vi "Software.Service.SNDB Communication Wrapper.vi"(0 "Log In Data":cluster{"Username":string, "Password":string}, 1 "Command":T1, 2 "Verify value":bool, 3 "File Path":string, 5 "Serial Number":string, 9 "Id(handle)":string, 11 "Error In (no error)":errorcluster, 12 "state":string, 13 "value":string) -> (4 "Operation Successful?":bool, 6 "UUT_Type":string, 10 "MAC_addresses":cluster{"MAC":string, "Status":string}[](array[cluster]), 15 "Error Out":errorcluster)   [LabVIEW 2026, in "Connect_to_SNDB_library.lvlib"]
uses:
  Connect_to_SNDB_library.lvlib
  Software.Service.SNDB Communication Wrapper Command.ctl
  Libray.Connect_to_SNDB_Command.ctl
  BB115/LabVIEW/Additional Libraries/Connect to SNDB Library.lvlibp/LabVIEW.Library/Libray.Connect_to_SNDB_Command.ctl
  <vilib>/JDP Science/JSONtext/Next JSON Value.vi
  <vilib>/JDP Science/JSONtext/String Subset.vi
  <vilib>/JDP Science/JSONtext/support/Strip Quotes and Unescape.vi
  <vilib>/JDP Science/JSONtext/Parsing/Advance past next JSON Value (inlined COPY).vi
  <vilib>/JDP Science/JSONtext/support/Unescape JSON string.vi
  <vilib>/JDP Science/JSONtext/Parsing/Advance past whitespace.vi
  <vilib>/JDP Science/JSONtext/Parsing/Advance past String.vi
  <vilib>/JDP Science/JSONtext/Parsing/Advance past Number.vi
  <vilib>/JDP Science/JSONtext/Parsing/Advance past Line Ending.vi
  <vilib>/JDP Science/JSONtext/Parsing/Parse Full Path or Item Name.vi
  <vilib>/JDP Science/JSONtext/Parsing/Advance past Array.vi
  <vilib>/JDP Science/JSONtext/Parsing/Advance past Object.vi
  <vilib>/JDP Science/JSONtext/support/Error Cluster From Code.vi
  <vilib>/JDP Science/JSONtext/Offset/Find Item Locations by Path.vi
  <vilib>/JDP Science/JSONtext/JSONtext.lvlib
  BB115/LabVIEW/Additional Libraries/Connect to SNDB Library.lvlibp
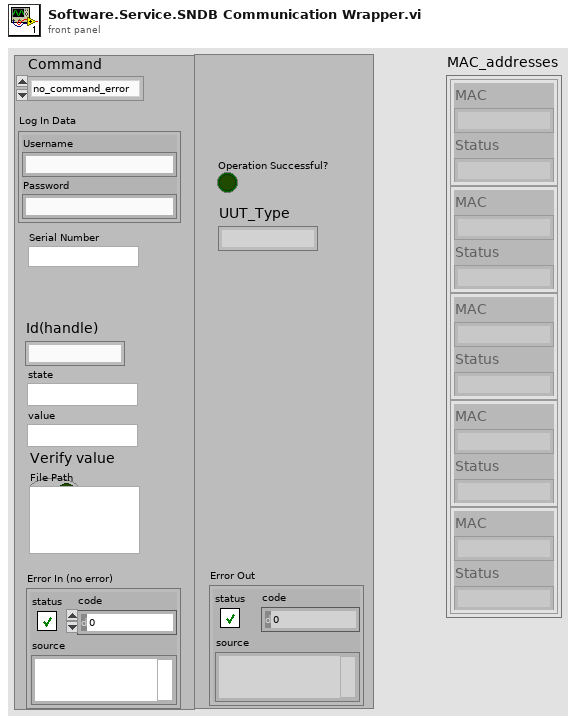
[diagram p1: front panel]
types:
  T1 = typedef "Connect_to_SNDB_library.lvlib/Software.Service.SNDB Communication Wrapper Command.ctl" = enum16{"no_command_error", "Initialize_Components_Login_Create_Token", "Get_UUT_Type", "Update steps", "Upload_PDF_Report", "Revoke_Token_Deinitialize_Components", "Reserve_MAC_addresses_for_a_Serial_Number", "Mark_a_reserved_MAC_address_as_flashed", "Get_all_MAC_addresses_for_a_Serial_Number", "Get_data_of_a_step"}
  T2 = typedef "Connect_to_SNDB_library.lvlib/Libray.Connect_to_SNDB_Command.ctl" = enum16{"No command", "Initialize HTTPS", "Authentication: Creat a token", "Authentication: Get all tokens", "Authentication: Revoke the token", "Label: Creat a label configuration", "Label: Get all configured labels", "Label: Update the label configuration", "Label: Delete the label configuration", "Label: Creat a colour ribbon", "Label: Update the colour ribbon", "Label: Get all colour ribbons", "Label: Delete the colour ribbon", "Label: Creat a label tape", "Label: Update the label tape", "Label: Get all label tapes", "Label: Delete the label tape", "Label: Get all label parameters", "Product: Get all product informations", "Product: Get all reading steps", "Seriennummer: Update the info text", "Seriennummer: Set all step states open", "Seriennummer: Update step states", "Seriennummer: Get data and steps", "Seriennummer: Get all label configurations", "Seriennummer: Create a text report(Prüfbericht)", "Seriennummer: Get the text report(Prüfbericht)", "Seriennummer: Delete the text report(Prüfbericht)", "Seriennummer: Upload a document(txt file)", "Seriennummer: Get the document", "Seriennummer: Get the document thumbnail", "Seriennummer: Delete the document", "Seriennummer: Bulk lookup", "Vorgang: Update the description text", "Vorgang: Migrate serial numbers to a Vorgang", "Vorgang: Migrate serial numbers to a product revision", "Vorgang: Update step states", "Vorgang: Create test reports(Prüfprotokoll)", "Vorgang: Get basic data", "Vorgang: Get serial number data and steps", "Vorgang: Get all serial numbers", "Vorgang: Generate a CSV file", "Vorgang: Generate an XLSX file", "Vorgang: Get a CSV file(Fertigmeldung report)", "Fertigmeldung: Create a Fertigmeldung", "Fertigmeldung: Revert the Fertigmeldung", "User: Get all users", "User: Update an user", "User: Get a single user", "User: Get all user roles", "User: Update a user role", "User: Get a single user role", "User: Get all permissions", "Search: Get Vorgang/Produkt combinations", "Search: Get Vorgang/Produkt/SN combinations", "Search: Get Seriennummern by Vorgang and Produkt", "Search: Lookup Vorgang", "MAC addresses: Get all reserved MAC addresses", "MAC addresses: Get the most recently reserved MAC addresses", "MAC addresses: Get data for a MAC address", "MAC addresses: Reserve a number of MAC addresses for a Seriennummer", "MAC addresses: Make a reserved MAC address as flashed", "Deinitialize HTTPs"}
  T3 = cluster{"stepType":string, "stepID":string, "state":string, "scannedValueOrChoice":string}
  T4 = typedef "Connect to SNDB Library.lvlibp/Libray.Connect_to_SNDB_Command.ctl" = enum16{"No command", "Initialize HTTPS", "Authentication: Creat a token", "Authentication: Get all tokens", "Authentication: Revoke the token", "Label: Creat a label configuration", "Label: Get all configured labels", "Label: Update the label configuration", "Label: Delete the label configuration", "Label: Creat a colour ribbon", "Label: Update the colour ribbon", "Label: Get all colour ribbons", "Label: Delete the colour ribbon", "Label: Creat a label tape", "Label: Update the label tape", "Label: Get all label tapes", "Label: Delete the label tape", "Label: Get all label parameters", "Product: Get all product informations", "Product: Get all reading steps", "Seriennummer: Update the info text", "Seriennummer: Set all step states open", "Seriennummer: Update step states", "Seriennummer: Get data and steps", "Seriennummer: Get all label configurations", "Seriennummer: Create a text report(Prüfbericht)", "Seriennummer: Get the text report(Prüfbericht)", "Seriennummer: Delete the text report(Prüfbericht)", "Seriennummer: Upload a document(txt file)", "Seriennummer: Get the document", "Seriennummer: Get the document thumbnail", "Seriennummer: Delete the document", "Seriennummer: Bulk lookup", "Vorgang: Update the description text", "Vorgang: Migrate serial numbers to a Vorgang", "Vorgang: Migrate serial numbers to a product revision", "Vorgang: Update step states", "Vorgang: Create test reports(Prüfprotokoll)", "Vorgang: Get basic data", "Vorgang: Get serial number data and steps", "Vorgang: Get all serial numbers", "Vorgang: Generate a CSV file", "Vorgang: Generate an XLSX file", "Vorgang: Get a CSV file(Fertigmeldung report)", "Fertigmeldung: Create a Fertigmeldung", "Fertigmeldung: Revert the Fertigmeldung", "User: Get all users", "User: Update an user", "User: Get a single user", "User: Get all user roles", "User: Update a user role", "User: Get a single user role", "User: Get all permissions", "Search: Get Vorgang/Produkt combinations", "Search: Get Vorgang/Produkt/SN combinations", "Search: Get Seriennummern by Vorgang and Produkt", "Search: Lookup Vorgang", "MAC addresses: Get all reserved MAC addresses", "MAC addresses: Get the most recently reserved MAC addresses", "MAC addresses: Get data for a MAC address", "MAC addresses: Reserve a number of MAC addresses for a Seriennummer", "MAC addresses: Make a reserved MAC address as flashed", "Deinitialize HTTPs"}
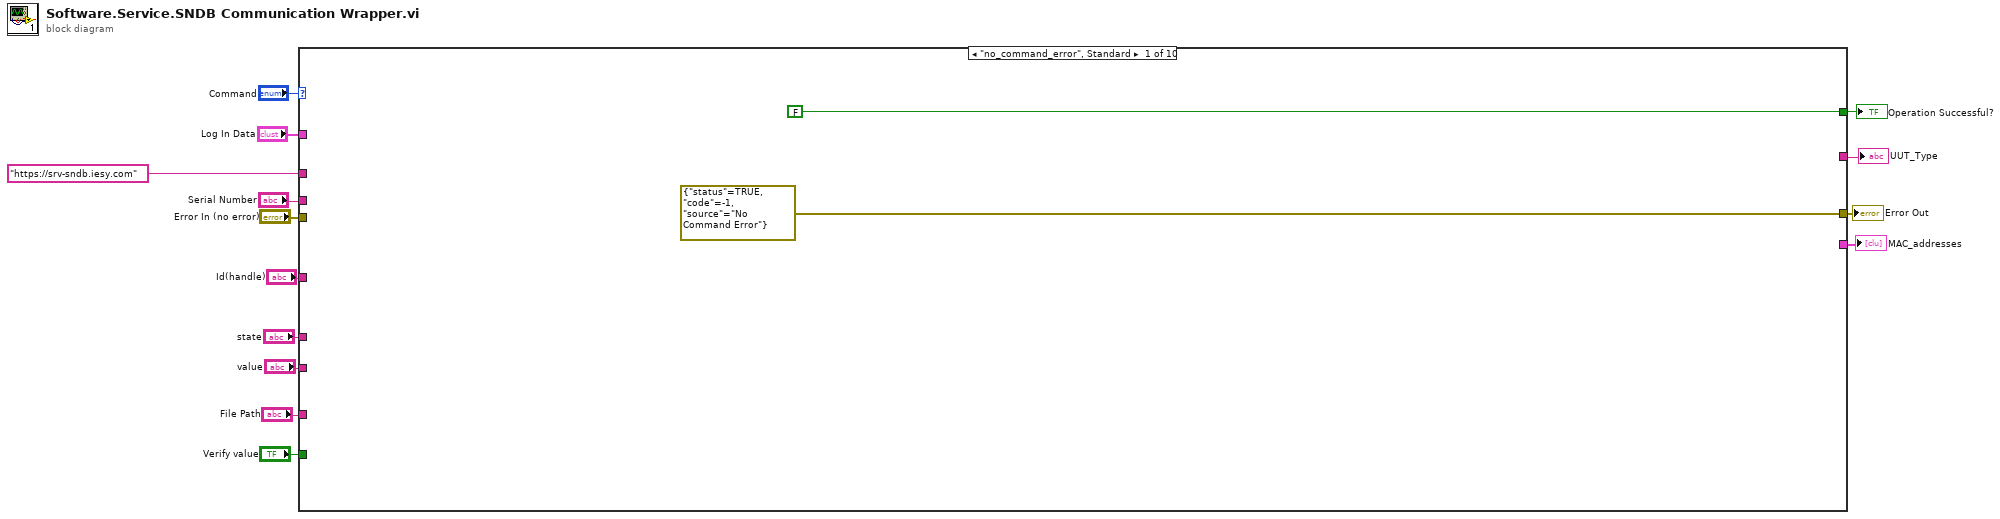
[diagram p0: block diagram]
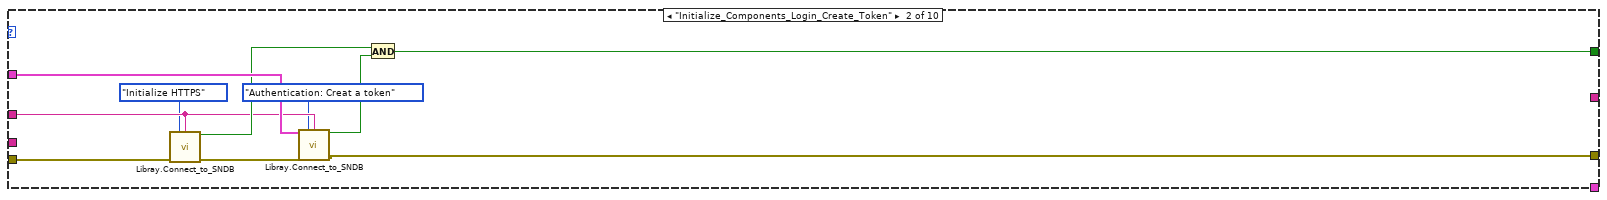
[diagram p2: hidden frame]
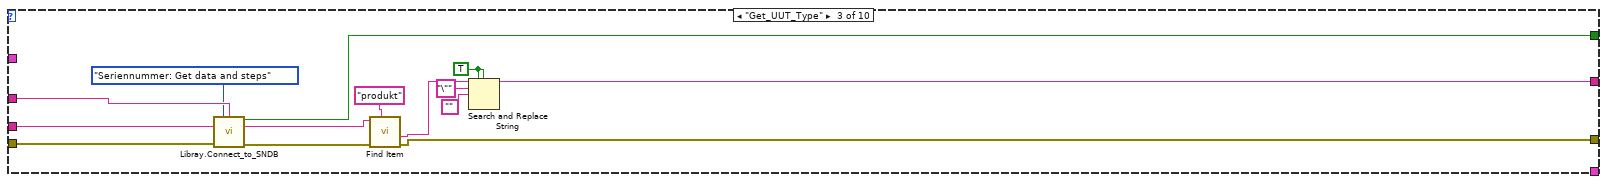
[diagram p3: hidden frame]
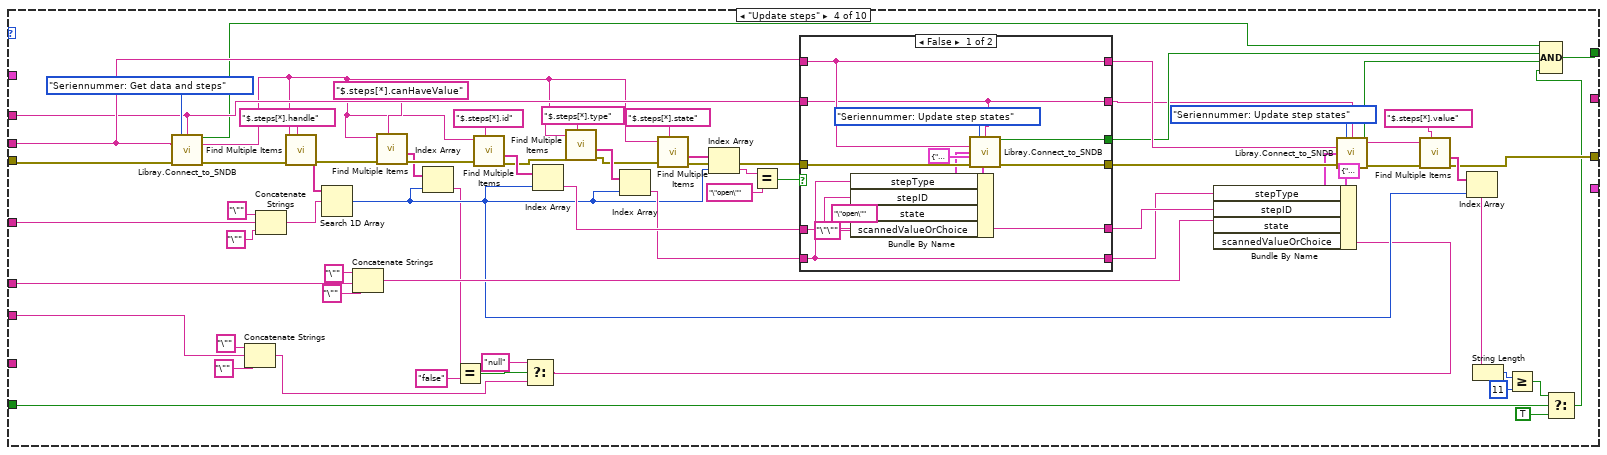
[diagram p4: hidden frame]
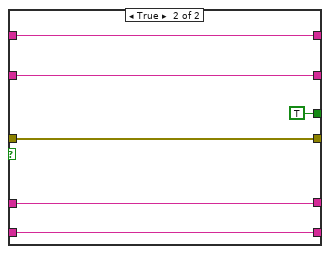
[diagram p5: hidden frame]
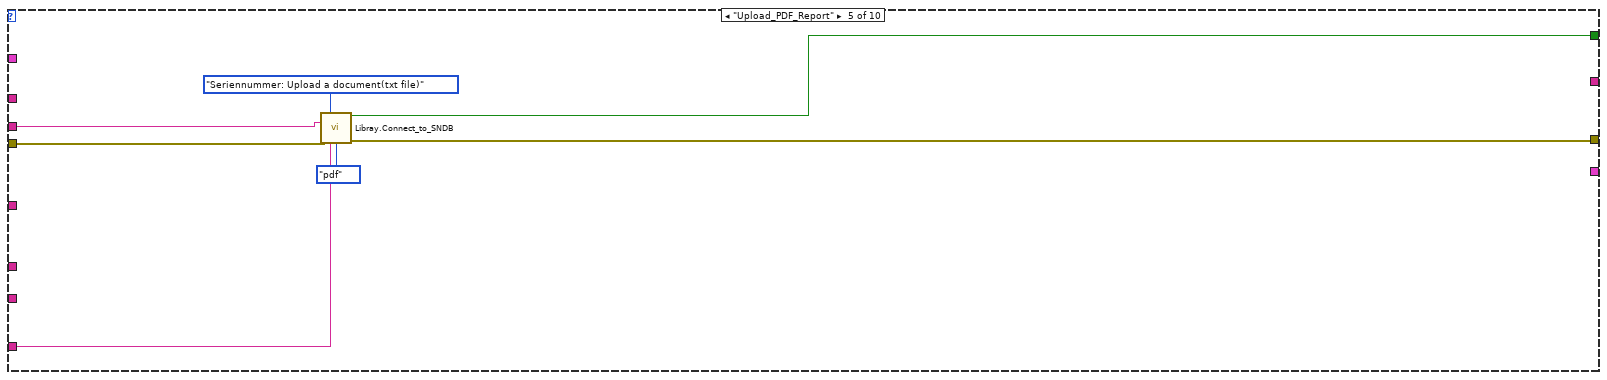
[diagram p6: hidden frame]
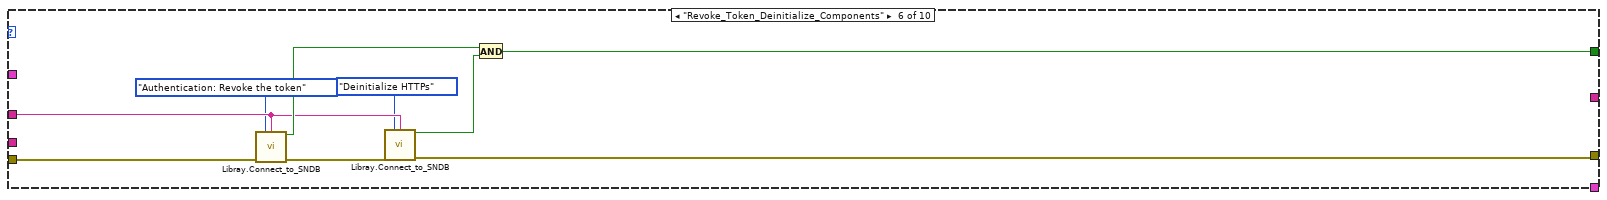
[diagram p7: hidden frame]
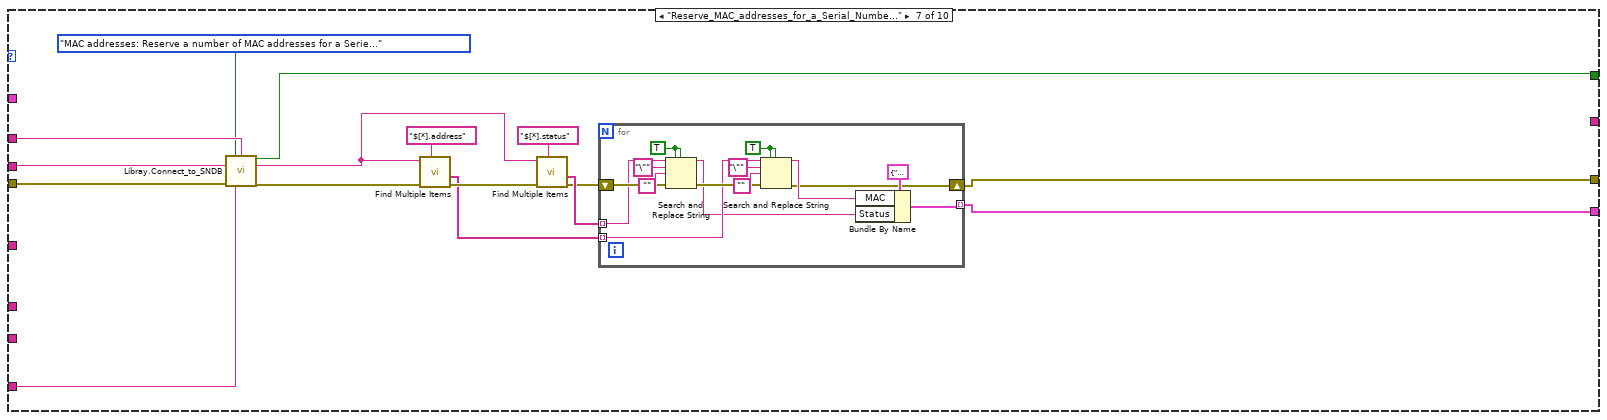
[diagram p8: hidden frame]
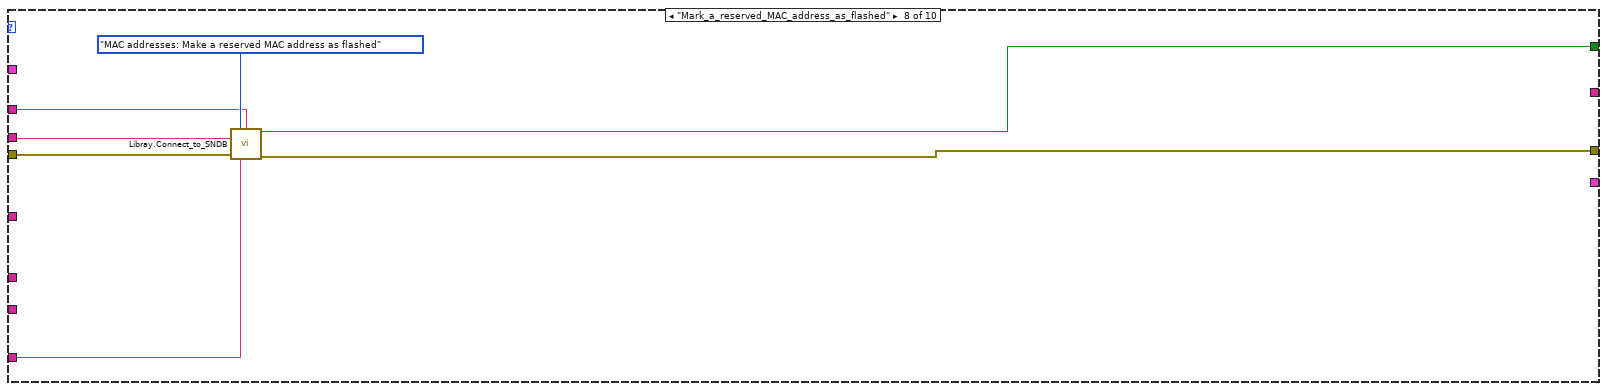
[diagram p9: hidden frame]
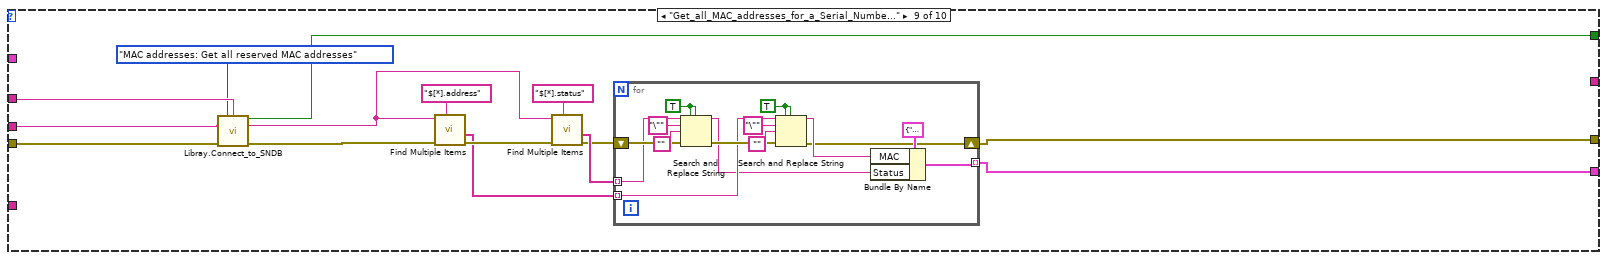
[diagram p10: hidden frame]
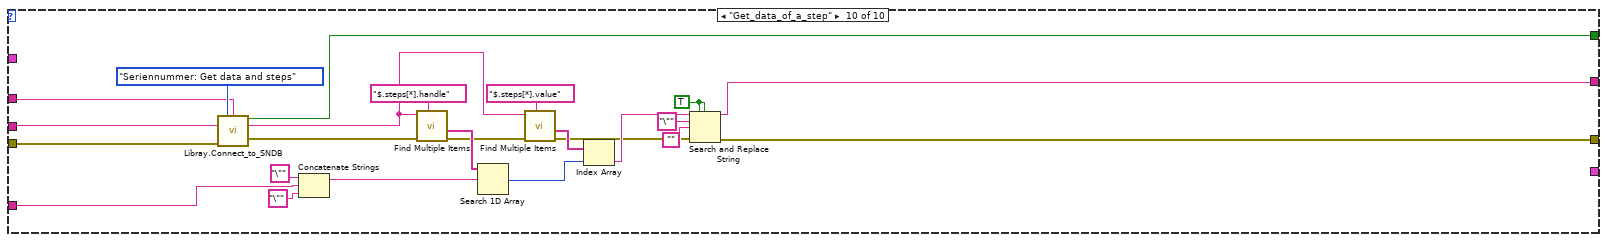
[diagram p11: hidden frame]
diagram:
  n1 = case shown="\"no_command_error\", Standard" "Command" {
    tunnel: [FALSE w26 w39 w91 w129 w139 w148 w176 w192 w215] -> w14
    tunnel: "Error In (no error)" -> [_ w25 w40 w59 w133 w141 w157 w180 w194 w233]
    tunnel: [errorcluster {"status"=TRUE, "code"=-1, "source"="No Command Error"} ("error out") w23 w36 w74 w130 w140 w144 w177 w182 w212] -> w12
    tunnel: "Log In Data" -> [_ w22 _ _ _ _ _ _ _ _]
    tunnel: [_ _ w30 _ _ _ _ _ _ w213] -> w9
    tunnel: "Serial Number" -> [_ _ w29 w58 w128 _ w155 w174 w183 w231]
    tunnel: "value" -> [_ _ _ w85 _ _ _ _ _ _]
    tunnel: "Id(handle)" -> [_ _ _ w88 _ _ _ _ _ w211]
    tunnel: "state" -> [_ _ _ w81 _ _ _ _ _ _]
    tunnel: "https://srv-sndb.iesy.com" ("Curl") -> [_ w19 w28 w56 _ w136 w158 w178 w195 w232]
    tunnel: "Verify value" -> [_ _ _ w68 _ _ _ _ _ _]
    tunnel: "File Path" -> [_ _ _ _ w131 _ w143 w175 _ _]
    tunnel: [_ _ _ _ _ _ w145 _ w181 _] -> w1
    frame "no_command_error", Default {
    }
    frame "Initialize_Components_Login_Create_Token" {
      n2 = call "Libray.Connect_to_SNDB.vi"("Command"=Libray.Connect_to_SNDB_Command."Initialize HTTPS", "Curl"=w19, "Fehler (Eingang, kein Fehler)"=w25) -> ("Successful?"=w21:bool, "error out"=w24:errorcluster)  [unwired: 9 in, 2 out]
      n3 = call "Libray.Connect_to_SNDB.vi"("Log In Data"=w22, "Command"=Libray.Connect_to_SNDB_Command."Authentication: Creat a token", "Curl"=w19, "Fehler (Eingang, kein Fehler)"=w24) -> ("Successful?"=w20:bool, "error out"=w23:errorcluster)  [unwired: 8 in, 2 out]
      n4 = And(x=w21, y=w20) -> (x .and. y?=w26:bool)
    }
    frame "Get_UUT_Type" {
      w34 = TRUE ("Alle ersetzen? (F)")
      n5 = call "Libray.Connect_to_SNDB.vi"("Command"=Libray.Connect_to_SNDB_Command."Seriennummer: Get data and steps", "Curl"=w28, "Serial Number"=w29, "Fehler (Eingang, kein Fehler)"=w40) -> ("Successful?"=w39:bool, "body"=w35:string, "error out"=w37:errorcluster)  [unwired: 8 in, 1 out]
      n6 = call <vilib>:"Find Item.vi"("$Path or Item Name"="produkt", "error in (no error)"=w37, "JSON"=w35) -> ("error out"=w36:errorcluster, "<JSON>"=w31:string)  [unwired: 5 in, 2 out]
      n7 = Search and Replace String(replace all?=w34, case sensitive?=w34, input string=w31, search string="\"" ("Such-String"), replace string="") -> (result string=w30:string)  [unwired: 3 in, 3 out]
    }
    frame "Update steps" {
      n8 = call "Libray.Connect_to_SNDB.vi"("Command"=Libray.Connect_to_SNDB_Command."Seriennummer: Get data and steps", "Curl"=w56, "Serial Number"=w58, "Fehler (Eingang, kein Fehler)"=w59) -> ("Successful?"=w55:bool, "body"=w41:string, "error out"=w54:errorcluster)  [unwired: 8 in, 1 out]
      n9 = Concatenate Strings("\"" ("String"), w85, "\"" ("String")) -> (w42:string)
      n10 = Concatenate Strings("\"" ("String"), w88, "\"" ("String")) -> (w89:string)
      n11 = call <vilib>:"Find Multiple Items.vi"("$Path or Item Name"="$.steps[*].handle", "error in (no error)"=w54, "JSON"=w41) -> ("error out"=w51:errorcluster, "<JSON>"=w107:string[])  [unwired: 5 in, 2 out]
      n12 = Search 1D Array(1D array=w107, element=w89) -> (index of element=w48:i32)  [unwired: 1 in]
      n13 = Concatenate Strings("\"" ("String"), w81, "\"" ("String")) -> (w82:string)
      n14 = call <vilib>:"Find Multiple Items.vi"("$Path or Item Name"="$.steps[*].canHaveValue", "error in (no error)"=w51, "JSON"=w41) -> ("error out"=w50:errorcluster, "<JSON>"=w49:string[])  [unwired: 5 in, 2 out]
      n15 = Index Array(array=w49, index=w48) -> (element=w47:string)
      n16 = Equal?(x=w47, y="false") -> (x = y?=w45:bool)
      n17 = call <vilib>:"Find Multiple Items.vi"("$Path or Item Name"="$.steps[*].id", "error in (no error)"=w50, "JSON"=w41) -> ("error out"=w64:errorcluster, "<JSON>"=w99:string[])  [unwired: 5 in, 2 out]
      n18 = Select(t="null" ("y"), s=w45, f=w42) -> (s? t:f=w44:string)
      n19 = Index Array(array=w99, index=w48) -> (element=w80:string)
      n20 = call <vilib>:"Find Multiple Items.vi"("$Path or Item Name"="$.steps[*].type", "error in (no error)"=w64, "JSON"=w41) -> ("error out"=w63:errorcluster, "<JSON>"=w65:string[])  [unwired: 5 in, 2 out]
      n21 = Index Array(array=w65, index=w48) -> (element=w62:string)
      n22 = call <vilib>:"Find Multiple Items.vi"("$Path or Item Name"="$.steps[*].state", "error in (no error)"=w63, "JSON"=w41) -> ("error out"=w101:errorcluster, "<JSON>"=w105:string[])  [unwired: 5 in, 2 out]
      n23 = Index Array(array=w105, index=w48) -> (element=w104:string)
      n24 = Equal?(x=w104, y="\"open\"") -> (x = y?=w102:bool)
      n25 = case shown="False" w102 {
        tunnel: w101 -> [w120 w125]
        tunnel: w58 -> [w115 w126]
        tunnel: w80 -> [w114 w124]
        tunnel: [w116 w125] -> w98
        tunnel: [w115 w126] -> w97
        tunnel: [w114 w124] -> w94
        tunnel: [w113 TRUE ("Successful?")] -> w93
        tunnel: w62 -> [w112 w122]
        tunnel: [w112 w122] -> w90
        tunnel: w56 -> [w111 w121]
        tunnel: [w111 w121] -> w79
        frame False {
          n26 = Bundle By Name(cluster=T3 {"stepType"="", "stepID"="", "state"="", "scannedValueOrChoice"=""} ("Update step"), "stepType"=w112, "stepID"=w114, "state"="\"open\"", "scannedValueOrChoice"="\"\"") -> (w118:T3)
          n27 = call "Libray.Connect_to_SNDB.vi"("Command"=Libray.Connect_to_SNDB_Command."Seriennummer: Update step states", "Curl"=w111, "Serial Number"=w115, "Update step"=w118, "Fehler (Eingang, kein Fehler)"=w120) -> ("Successful?"=w113:bool, "error out"=w116:errorcluster)  [unwired: 7 in, 2 out]
        }
        frame True {
        }
      }
      n28 = Bundle By Name(cluster=T3 {"stepType"="", "stepID"="", "state"="", "scannedValueOrChoice"=""} ("Update step"), "stepType"=w90, "stepID"=w94, "state"=w82, "scannedValueOrChoice"=w44) -> (w95:T3)
      n29 = call "Libray.Connect_to_SNDB.vi"("Command"=Libray.Connect_to_SNDB_Command."Seriennummer: Update step states", "Curl"=w79, "Serial Number"=w97, "Update step"=w95, "Fehler (Eingang, kein Fehler)"=w98) -> ("Successful?"=w92:bool, "body"=w77:string, "error out"=w75:errorcluster)  [unwired: 7 in, 1 out]
      n30 = call <vilib>:"Find Multiple Items.vi"("$Path or Item Name"="$.steps[*].value", "error in (no error)"=w75, "JSON"=w77) -> ("error out"=w74:errorcluster, "<JSON>"=w76:string[])  [unwired: 5 in, 2 out]
      n31 = Index Array(array=w76, index=w48) -> (element=w73:string)
      n32 = String Length(string=w73) -> (length=w72:i32)
      n33 = Greater Or Equal?(x=w72, y=11) -> (x >= y?=w70:bool)
      n34 = Select(t=w70, s=w68, f=TRUE) -> (s? t:f=w69:bool)
      n35 = Compound Arithmetic op=AND ("Mehrfacharithmetik")(w55, w93, w92, w69) -> (w91:bool)
    }
    frame "Upload_PDF_Report" {
      n36 = call "Libray.Connect_to_SNDB.vi"("Command"=Libray.Connect_to_SNDB_Command."Seriennummer: Upload a document(txt file)", "Serial Number"=w128, "Fehler (Eingang, kein Fehler)"=w133, "Input String"=w131, "Type of the uploaded file"=enum16{"txt", "pdf", "image/jpeg"}."pdf") -> ("Successful?"=w129:bool, "error out"=w130:errorcluster)  [unwired: 7 in, 2 out]
    }
    frame "Revoke_Token_Deinitialize_Components" {
      n37 = call "Libray.Connect_to_SNDB.vi"("Command"=Libray.Connect_to_SNDB_Command."Authentication: Revoke the token", "Curl"=w136, "Fehler (Eingang, kein Fehler)"=w141) -> ("Successful?"=w138:bool, "error out"=w142:errorcluster)  [unwired: 9 in, 2 out]
      n38 = call "Libray.Connect_to_SNDB.vi"("Command"=Libray.Connect_to_SNDB_Command."Deinitialize HTTPs", "Curl"=w136, "Fehler (Eingang, kein Fehler)"=w142) -> ("Successful?"=w137:bool, "error out"=w140:errorcluster)  [unwired: 9 in, 2 out]
      n39 = And(x=w138, y=w137) -> (x .and. y?=w139:bool)
    }
    frame "Reserve_MAC_addresses_for_a_Serial_Number" {
      n40 = call "Libray.Connect_to_SNDB.vi"("Command"=Libray.Connect_to_SNDB_Command."MAC addresses: Reserve a number of MAC addresses for a Seriennummer", "Curl"=w158, "Serial Number"=w155, "Fehler (Eingang, kein Fehler)"=w157, "Input String"=w143) -> ("Successful?"=w148:bool, "body"=w147:string, "error out"=w146:errorcluster)  [unwired: 7 in, 1 out]
      n41 = call <vilib>:"Find Multiple Items.vi"("$Path or Item Name"="$[*].address", "error in (no error)"=w146, "JSON"=w147) -> ("error out"=w152:errorcluster, "<JSON>"=w151:string[])  [unwired: 5 in, 2 out]
      n42 = call <vilib>:"Find Multiple Items.vi"("$Path or Item Name"="$[*].status", "error in (no error)"=w152, "JSON"=w147) -> ("error out"=w149:errorcluster, "<JSON>"=w150:string[])  [unwired: 5 in, 2 out]
      n43 = for {
        tunnel: w151 -> [w165] mode=indexing
        tunnel: w150 -> [w164] mode=indexing
        tunnel: [w160] -> w145 mode=indexing
        shift-right: [w159] -> w144
        shift-left: w149 -> [w170]
        w169 = TRUE ("Alle ersetzen? (F)")
        w171 = TRUE ("Alle ersetzen? (F)")
        n44 = Search and Replace String(replace all?=w171, case sensitive?=w171, input string=w164, search string="\"" ("Such-String"), replace string="", error in=w170) -> (result string=w161:string, error out=w166:errorcluster)  [unwired: 2 in, 2 out]
        n45 = Search and Replace String(replace all?=w169, case sensitive?=w169, input string=w165, search string="\"" ("Such-String"), replace string="", error in=w166) -> (result string=w162:string, error out=w159:errorcluster)  [unwired: 2 in, 2 out]
        n46 = Bundle By Name(cluster=cluster{"MAC":string, "Status":string} {"MAC"="", "Status"=""}, "MAC"=w162, "Status"=w161) -> (w160:cluster{"MAC":string, "Status":string})
      }
    }
    frame "Mark_a_reserved_MAC_address_as_flashed" {
      n47 = call "Libray.Connect_to_SNDB.vi"("Command"=Libray.Connect_to_SNDB_Command."MAC addresses: Make a reserved MAC address as flashed", "Curl"=w178, "Serial Number"=w174, "Fehler (Eingang, kein Fehler)"=w180, "Input String"=w175) -> ("Successful?"=w176:bool, "error out"=w177:errorcluster)  [unwired: 7 in, 2 out]
    }
    frame "Get_all_MAC_addresses_for_a_Serial_Number" {
      n48 = call "Libray.Connect_to_SNDB.vi"("Command"=Libray.Connect_to_SNDB_Command."MAC addresses: Get all reserved MAC addresses", "Curl"=w195, "Serial Number"=w183, "Fehler (Eingang, kein Fehler)"=w194) -> ("Successful?"=w192:bool, "body"=w184:string, "error out"=w185:errorcluster)  [unwired: 8 in, 1 out]
      n49 = call <vilib>:"Find Multiple Items.vi"("$Path or Item Name"="$[*].address", "error in (no error)"=w185, "JSON"=w184) -> ("error out"=w189:errorcluster, "<JSON>"=w188:string[])  [unwired: 5 in, 2 out]
      n50 = call <vilib>:"Find Multiple Items.vi"("$Path or Item Name"="$[*].status", "error in (no error)"=w189, "JSON"=w184) -> ("error out"=w186:errorcluster, "<JSON>"=w187:string[])  [unwired: 5 in, 2 out]
      n51 = for {
        tunnel: w188 -> [w202] mode=indexing
        tunnel: w187 -> [w201] mode=indexing
        tunnel: [w197] -> w181 mode=indexing
        shift-right: [w196] -> w182
        shift-left: w186 -> [w207]
        w206 = TRUE ("Alle ersetzen? (F)")
        w208 = TRUE ("Alle ersetzen? (F)")
        n52 = Search and Replace String(replace all?=w208, case sensitive?=w208, input string=w201, search string="\"" ("Such-String"), replace string="", error in=w207) -> (result string=w198:string, error out=w203:errorcluster)  [unwired: 2 in, 2 out]
        n53 = Search and Replace String(replace all?=w206, case sensitive?=w206, input string=w202, search string="\"" ("Such-String"), replace string="", error in=w203) -> (result string=w199:string, error out=w196:errorcluster)  [unwired: 2 in, 2 out]
        n54 = Bundle By Name(cluster=cluster{"MAC":string, "Status":string} {"MAC"="", "Status"=""}, "MAC"=w199, "Status"=w198) -> (w197:cluster{"MAC":string, "Status":string})
      }
    }
    frame "Get_data_of_a_step" {
      w222 = TRUE ("Alle ersetzen? (F)")
      n55 = call "Libray.Connect_to_SNDB.vi"("Command"=Libray.Connect_to_SNDB_Command."Seriennummer: Get data and steps", "Curl"=w232, "Serial Number"=w231, "Fehler (Eingang, kein Fehler)"=w233) -> ("Successful?"=w215:bool, "body"=w214:string, "error out"=w216:errorcluster)  [unwired: 8 in, 1 out]
      n56 = Concatenate Strings("\"" ("String"), w211, "\"" ("String")) -> (w217:string)
      n57 = call <vilib>:"Find Multiple Items.vi"("$Path or Item Name"="$.steps[*].handle", "error in (no error)"=w216, "JSON"=w214) -> ("error out"=w226:errorcluster, "<JSON>"=w229:string[])  [unwired: 5 in, 2 out]
      n58 = Search 1D Array(1D array=w229, element=w217) -> (index of element=w225:i32)  [unwired: 1 in]
      n59 = call <vilib>:"Find Multiple Items.vi"("$Path or Item Name"="$.steps[*].value", "error in (no error)"=w226, "JSON"=w214) -> ("error out"=w220:errorcluster, "<JSON>"=w227:string[])  [unwired: 5 in, 2 out]
      n60 = Index Array(array=w227, index=w225) -> (element=w221:string)
      n61 = Search and Replace String(replace all?=w222, case sensitive?=w222, input string=w221, search string="\"" ("Such-String"), replace string="", error in=w220) -> (result string=w213:string, error out=w212:errorcluster)  [unwired: 2 in, 2 out]
    }
  }
  "Error Out" <- w12
  "Operation Successful?" <- w14
  "UUT_Type" <- w9
  "MAC_addresses" <- w1
